vi "Util_Trajectory_WriteFile_PathFinder.vi"(6 "Trajectory Is Relative":bool, 7 "UTIL_PATHFINDER_CONFIG":T7 {"ActualMaxVelocity-inches per sec" format="%21.5f"; "WheelbaseDepth-inches" format="%21.5f"; "WheelbaseWidth-inches" format="%21.5f"; "TimeDelta-Seconds" format="%21.5f"; "MaxJerk--Inches per sec2" format="%21.5f"; "MaxAcceleration - inches per sec2" format="%21.5f"; "PathMaxVelocity - inches per sec" format="%21.5f"}, 8 "UtilityWayPoints":T6[](array[typedef]) {"ANGLE" format="%13.3f"; "Y" format="%13.3f"; "X" format="%13.3f"}, 9 "TRAJECTORY":T1 {"States"."POSE"."ROTATION"."SIN" format="%13.4f"; "States"."POSE"."ROTATION"."COS" format="%13.4f"; "States"."POSE"."ROTATION"."VALUE" format="%13.4f"; "States"."POSE"."TRANSLATION"."Y" format="%14.3f"; "States"."POSE"."TRANSLATION"."X" format="%14.3f"; "TotalTImeSecs" format="%20.3f"}, 10 "Comment":string, 11 "Trajectory File Name":path) -> (0 "error out":errorcluster)   [LabVIEW 2019, in "Trajectory_Library.lvlib"]
doc: "Create a CSV file from a Trajectory data structure. This can be used on a PC or the RoboRIO. This is a customized version for Pathfinder created trajectories.\n\nParameters:\n - Trajectory - Data structure containing trajectory\n - PathfinderConfig - Data structure with pathfinder configuration.\n - Trajectory File Name - File name to write to. Existing files are overwritten.\n - Comment - Comment string to include in file comments.\n - Waypoints - waypoints to include in file comments\n - TrajectoryIsRelative - Relative if TRUE otherwise absolute.\n\nReturns:\n - Error out - returned error cluster"
uses:
  Trajectory_Library.lvlib
  TypeDef/DISPLAY_WEIGHTED_WAYPOINT.ctl
  TypeDef/TRANSLATION2D.ctl
  TypeDef/DISPLAY_WAYPOINT.ctl
  TypeDef/UTIL_PATHFINDER_CONFIG.ctl
  TypeDef/ROTATION2D.ctl
  TypeDef/POSE2D.ctl
  TypeDef/TRAJ_STATE.ctl
  TypeDef/TRAJECTORY.ctl
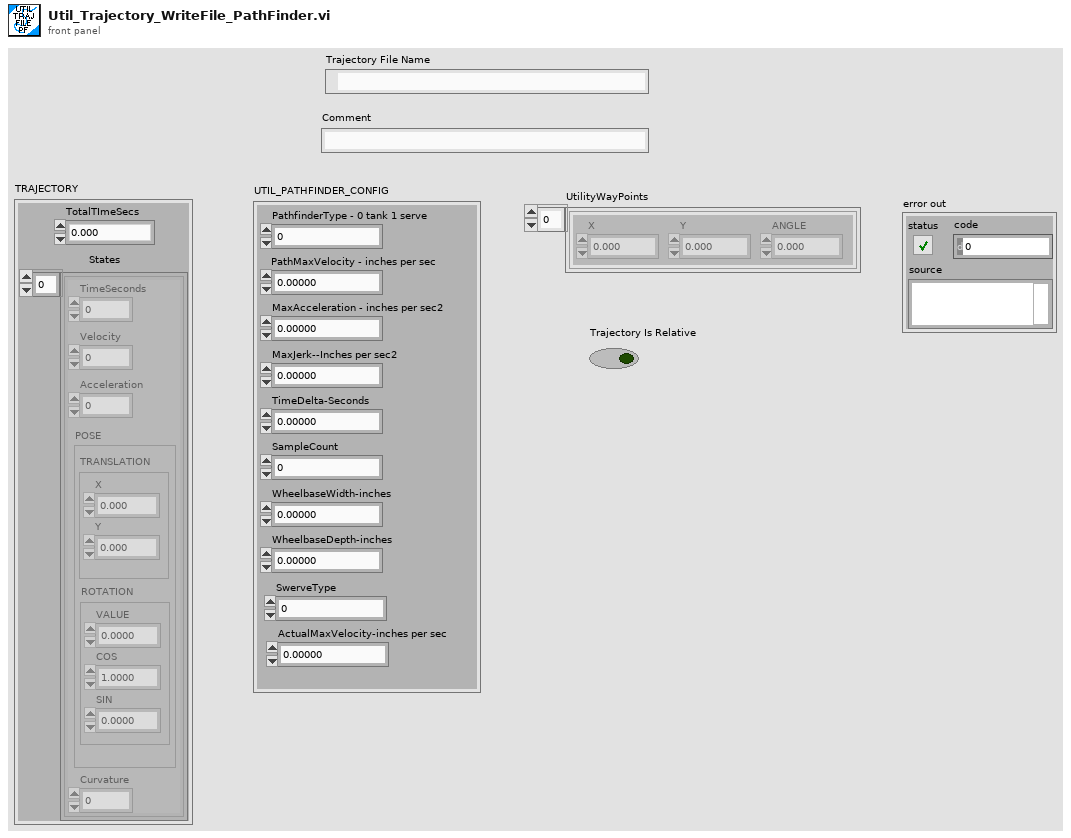
[diagram p1: front panel]
types:
  T1 = typedef "Trajectory_Library.lvlib/TRAJECTORY.ctl" = cluster{"TotalTImeSecs":dbl, "States":T2[]}
  T2 = typedef "Trajectory_Library.lvlib/TRAJ_STATE.ctl" = cluster{"TimeSeconds":dbl, "Velocity":dbl, "Acceleration":dbl, "POSE":T3, "Curvature":dbl}
  T3 = typedef "Trajectory_Library.lvlib/POSE2D.ctl" = cluster{"TRANSLATION":T4, "ROTATION":T5}
  T4 = typedef "Trajectory_Library.lvlib/TRANSLATION2D.ctl" = cluster{"X":dbl, "Y":dbl}
  T5 = typedef "Trajectory_Library.lvlib/ROTATION2D.ctl" = cluster{"VALUE":dbl, "COS":dbl, "SIN":dbl}
  T6 = typedef "Trajectory_Library.lvlib/DISPLAY_WAYPOINT.ctl" = cluster{"X":dbl, "Y":dbl, "ANGLE":dbl}
  T7 = typedef "Trajectory_Library.lvlib/UTIL_PATHFINDER_CONFIG.ctl" = cluster{"PathfinderType - 0 tank 1 serve":i32, "PathMaxVelocity - inches per sec":dbl, "MaxAcceleration - inches per sec2":dbl, "MaxJerk--Inches per sec2":dbl, "TimeDelta-Seconds":dbl, "SampleCount":i32, "WheelbaseWidth-inches":dbl, "WheelbaseDepth-inches":dbl, "SwerveType":i32, "ActualMaxVelocity-inches per sec":dbl}
  T8 = enum16{"open", "replace", "create", "open or create", "replace or create", "replace or create with confirmation"}
  T9 = typedef "Trajectory_Library.lvlib/DISPLAY_WEIGHTED_WAYPOINT.ctl" = cluster{"X":dbl, "Y":dbl, "ANGLE":dbl, "WEIGHT":dbl}
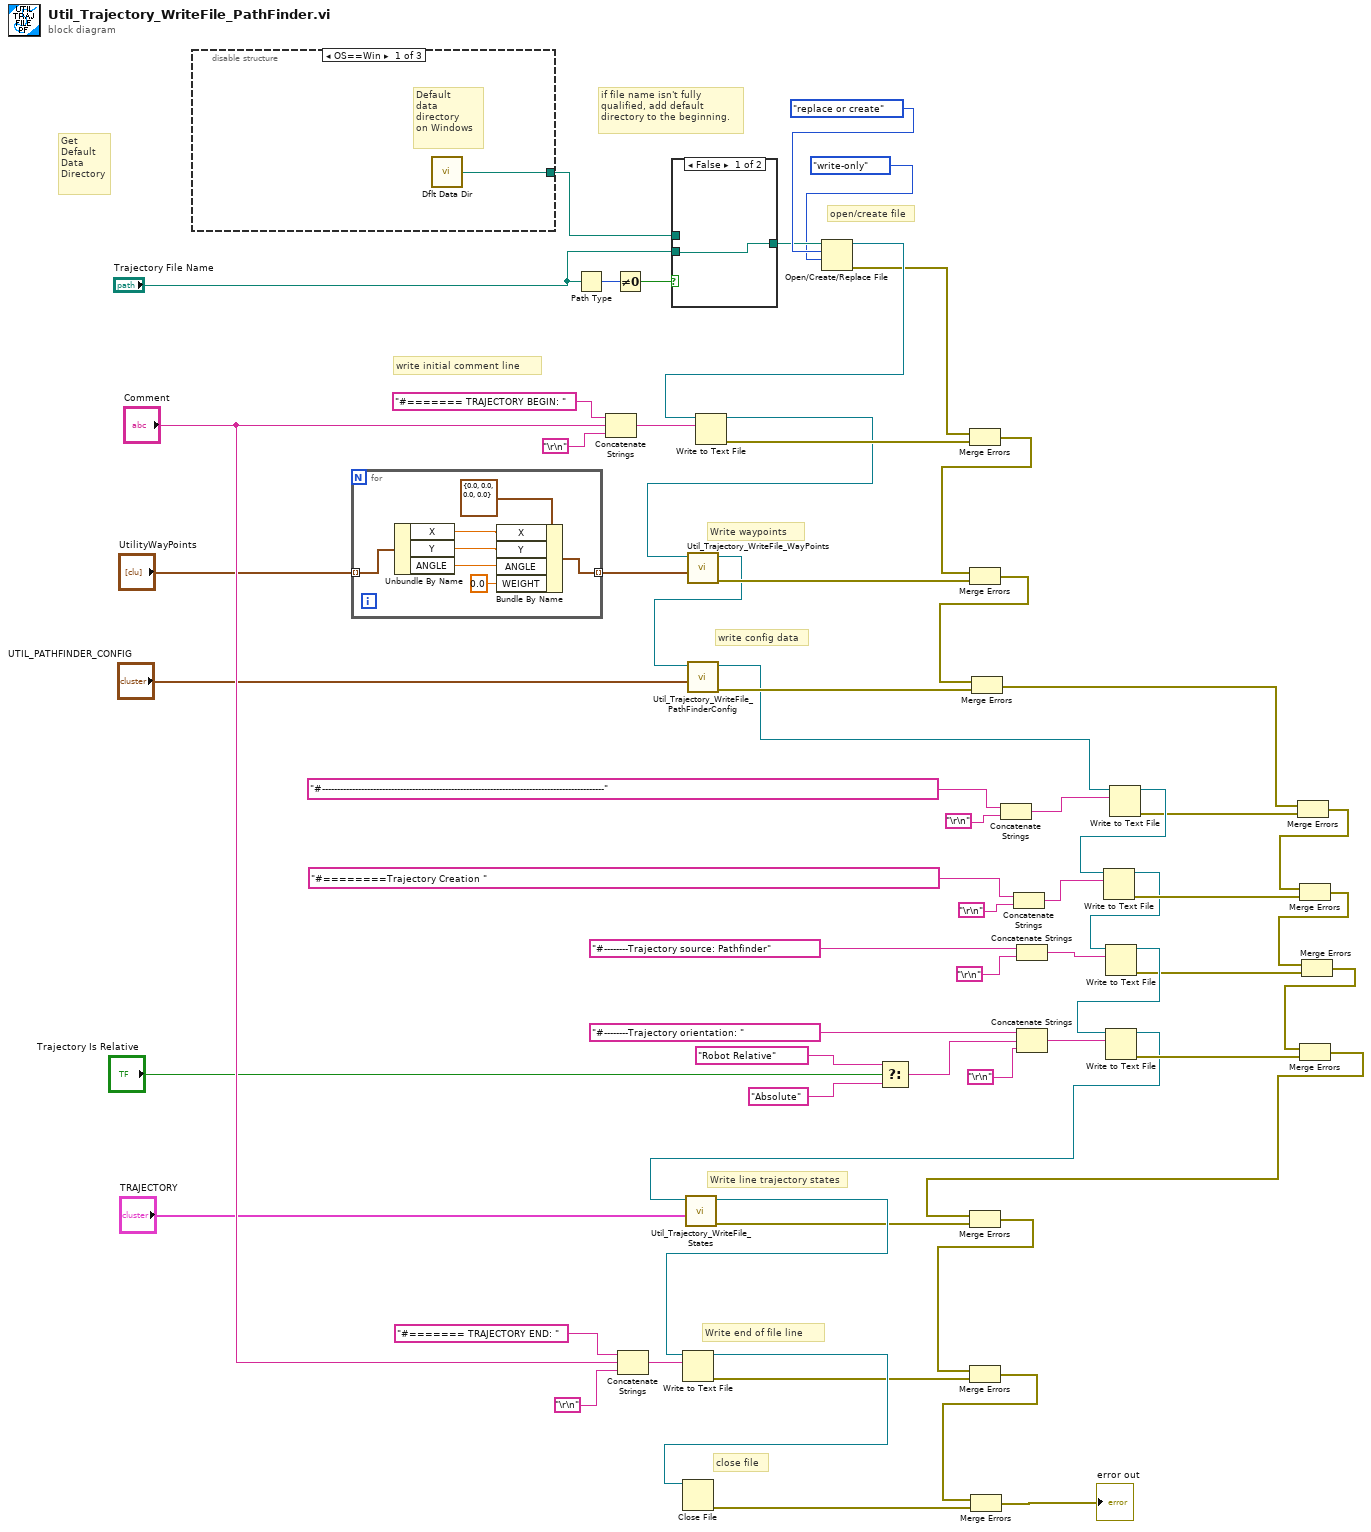
[diagram p0: block diagram]
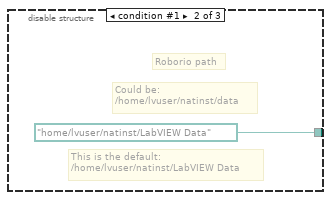
[diagram p2: hidden frame]
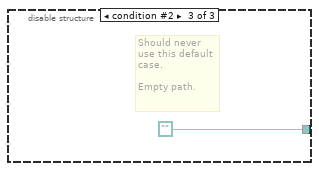
[diagram p3: hidden frame]
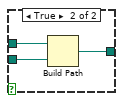
[diagram p4: hidden frame]
diagram:
  # "write config data"
  # "Write line trajectory states"
  # "open/create file"
  # "if file name isn't fully \nqualified, add default\ndirectory to the beginning."
  # "Get\nDefault\nData\nDirectory"
  # "Write waypoints"
  # "close file"
  # "Write end of file line"
  # "write initial comment line"
  n1 = disable-structure shown="OS==Win" {
    disable-tunnel: [w66 path "/home/lvuser/natinst/LabVIEW Data" path ""] -> w55
    frame condition #0 (active) {
      # "Default\ndata\ndirectory\non Windows"
      n2 = call <vilib>:"Dflt Data Dir.vi"() -> ("App:Default Data Directory"=w66:path)
    }
    frame condition #1 {
      # "This is the default:\n/home/lvuser/natinst/LabVIEW Data"
      # "Could be:\n/home/lvuser/natinst/data"
      # "Roborio path"
    }
    frame condition #2 {
      # "Should never\nuse this default\ncase.\n\nEmpty path."
    }
  }
  n3 = for {
    tunnel: "UtilityWayPoints" -> [w74] mode=indexing
    tunnel: [w69] -> w1 mode=indexing
    n4 = Unbundle By Name(w74) -> ("X"=w73:dbl, "Y"=w72:dbl, "ANGLE"=w71:dbl)
    n5 = Bundle By Name(cluster=T9 {"X"=0.0, "Y"=0.0, "ANGLE"=0.0, "WEIGHT"=0.0} ("UTIL_WEIGHTED_WAYPOINT"), "X"=w73, "Y"=w72, "ANGLE"=w71, "WEIGHT"=0.0) -> (w69:T9)
  }
  n6 = Path Type(1:"Trajectory File Name") -> (0:w58:i16)
  n7 = Concatenate Strings("#======= TRAJECTORY BEGIN: " ("string"), "Comment", "\r\n") -> (w63:string)
  n8 = Not Equal To 0?(x=w58) -> (x != 0?=w57:bool)
  n9 = Concatenate Strings("#======= TRAJECTORY END: " ("string"), "Comment", "\r\n") -> (w59:string)
  n10 = case shown="False" w57 {
    tunnel: [w76 w79] -> w54
    tunnel: w55 -> [_ w78]
    tunnel: "Trajectory File Name" -> [w76 w77]
    frame False {
    }
    frame True {
      n11 = Build Path(base path=w78, name or relative path=w77) -> (appended path=w79:path)
    }
  }
  n12 = Open/Create/Replace File(file path (use dialog)=w54, operation (0:open)=T8."replace or create", access (0:read/write)=enum16{"read/write", "read-only", "write-only"}."write-only") -> (refnum out=w52:refnum<file>, error out=w47:errorcluster)  [unwired: 3 in, 1 out]
  n13 = Write to Text File(file (use dialog)=w52, text=w63) -> (refnum out=w38:refnum<file>, error out=w48:errorcluster)  [unwired: 2 in, 1 out]
  n14 = call "Util_Trajectory_WriteFile_WayPoints.vi"("UtilityWayPoints"=w1, "Byte Steam File In"=w38) -> ("error out"=w46:errorcluster, "Byte Steam File Out"=w37:refnum<file>)  [unwired: 8 in]
  n15 = call "Util_Trajectory_WriteFile_PathFinderConfig.vi"("UTIL_PATHFINDER_CONFIG"="UTIL_PATHFINDER_CONFIG", "Byte Steam File In"=w37) -> ("error out"=w36:errorcluster, "Byte Steam File Out"=w17:refnum<file>)  [unwired: 8 in]
  n16 = Select(t="Robot Relative" ("string"), s="Trajectory Is Relative", f="Absolute" ("string")) -> (s? t:f=w25:string)
  n17 = Merge Errors(w47, w48) -> (w39:errorcluster)
  n18 = Merge Errors(w39, w46) -> (w35:errorcluster)
  n19 = Merge Errors(w35, w36) -> (w14:errorcluster)
  n20 = Concatenate Strings("#----------------------------------------------------------------------------------------------" ("string"), "\r\n") -> (w29:string)
  n21 = Concatenate Strings("#========Trajectory Creation " ("string"), "\r\n") -> (w32:string)
  n22 = Concatenate Strings("#--------Trajectory source: Pathfinder" ("string"), "\r\n") -> (w12:string)
  n23 = Concatenate Strings("#--------Trajectory orientation: " ("string"), w25, "\r\n") -> (w27:string)
  n24 = Write to Text File(file (use dialog)=w17, text=w29) -> (refnum out=w21:refnum<file>, error out=w19:errorcluster)  [unwired: 2 in, 1 out]
  n25 = Write to Text File(file (use dialog)=w21, text=w32) -> (refnum out=w9:refnum<file>, error out=w20:errorcluster)  [unwired: 2 in, 1 out]
  n26 = Write to Text File(file (use dialog)=w9, text=w12) -> (refnum out=w8:refnum<file>, error out=w7:errorcluster)  [unwired: 2 in, 1 out]
  n27 = Write to Text File(file (use dialog)=w8, text=w27) -> (refnum out=w16:refnum<file>, error out=w26:errorcluster)  [unwired: 2 in, 1 out]
  n28 = call "Util_Trajectory_WriteFile_States.vi"("Trajectory"="TRAJECTORY", "Byte Steam File In"=w16) -> ("error out"=w45:errorcluster, "Byte Steam File Out"=w50:refnum<file>)  [unwired: 8 in]
  n29 = Write to Text File(file (use dialog)=w50, text=w59) -> (refnum out=w49:refnum<file>, error out=w43:errorcluster)  [unwired: 2 in, 1 out]
  n30 = Close File(refnum=w49) -> (error out=w42:errorcluster)  [unwired: 1 in, 1 out]
  n31 = Merge Errors(w14, w19) -> (w18:errorcluster)
  n32 = Merge Errors(w18, w20) -> (w6:errorcluster)
  n33 = Merge Errors(w6, w7) -> (w5:errorcluster)
  n34 = Merge Errors(w5, w26) -> (w13:errorcluster)
  n35 = Merge Errors(w13, w45) -> (w44:errorcluster)
  n36 = Merge Errors(w44, w43) -> (w41:errorcluster)
  n37 = Merge Errors(w41, w42) -> (→"error out":errorcluster)
